vi "Measurement Logic.vi"(8 "error in":errorcluster, 9 "measurement configuration":T2={"Input Terminal Name"="Lorem ipsum dolor sit", "Counter Interface"="", "Active Edge"=10171, "Pulses"=0, "Timeout (s)"=0, "DUT Pin"=""} {"Active Edge" items=["Rising"=10280, "Falling"=10171]}, 10 "measure call context in":refnum<class "Measure Call Context.lvclass">) -> (0 "error out":errorcluster, 1 "Measurements Resuts":T1, 2 "measure call context out":refnum<class "Measure Call Context.lvclass">)   [LabVIEW 2025, in "Count Edges.lvclass"]
doc: "Contains the core logic for executing the measurement."
uses:
  Count Edges.lvclass
  <vilib>/Plug-In SDKs/Measurements/Measure Call Context/Measure Call Context.lvclass
  Measurement Configuration.ctl
  Measurement Results.ctl
  <vilib>/DAQmx/read.llb/DAQmx Read (Counter U32 1Chan 1Samp).vi
  <vilib>/DAQmx/create/channels.llb/DAQmx Create Channel (CI-Count Edges).vi
  <vilib>/DAQmx/miscellaneous.llb/DAQmx Fill In Error Info.vi
  <extravilib>/ChannelInstances/Event Messenger-bool/Instantiate.vi
  <resource>/objmgr/daqmx.rc
  <vilib>/Plug-In SDKs/Clients/Session Management V1/Session Reservation/Session Reservation.lvclass
  session-management/daqmxCounter/Session Management daqmxCounter.lvlib
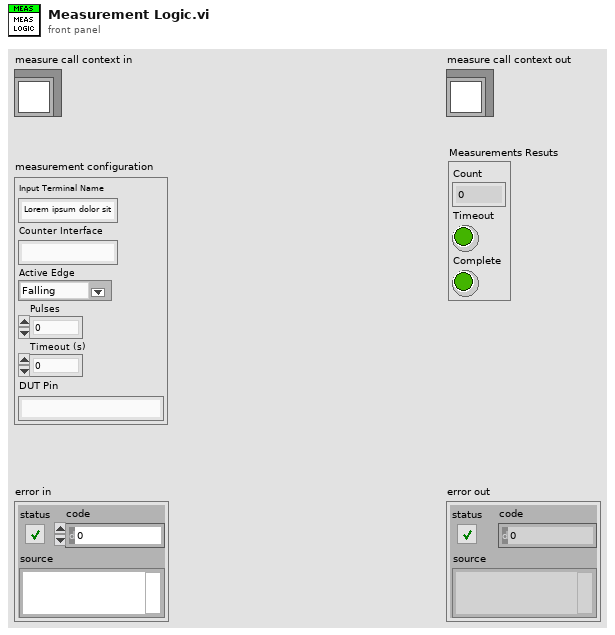
[diagram p1: front panel]
types:
  T1 = typedef "Count Edges.lvclass/Measurement Results.ctl" = cluster{"Count":u32, "Timeout":bool, "Complete":bool}
  T2 = typedef "Count Edges.lvclass/Measurement Configuration.ctl" = cluster{"Input Terminal Name":string, "Counter Interface":string, "Active Edge":i32, "Pulses":u32, "Timeout (s)":u32, "DUT Pin":string}
  T3 = typedef "Session Management daqmxCounter.lvlib/Connection with Session.ctl" = cluster{"connection":T4, "session":string}
  T4 = typedef "NI Session Management V1 Client.lvlib/Session Reservation.lvclass/Connection.ctl" = cluster{"pin or relay name":string, "site":i32, "instrument type id":string, "channel":string}
  T5 = typedef "Event Messenger-bool.lvlib/))Channel.ctl" = refnum<queue>
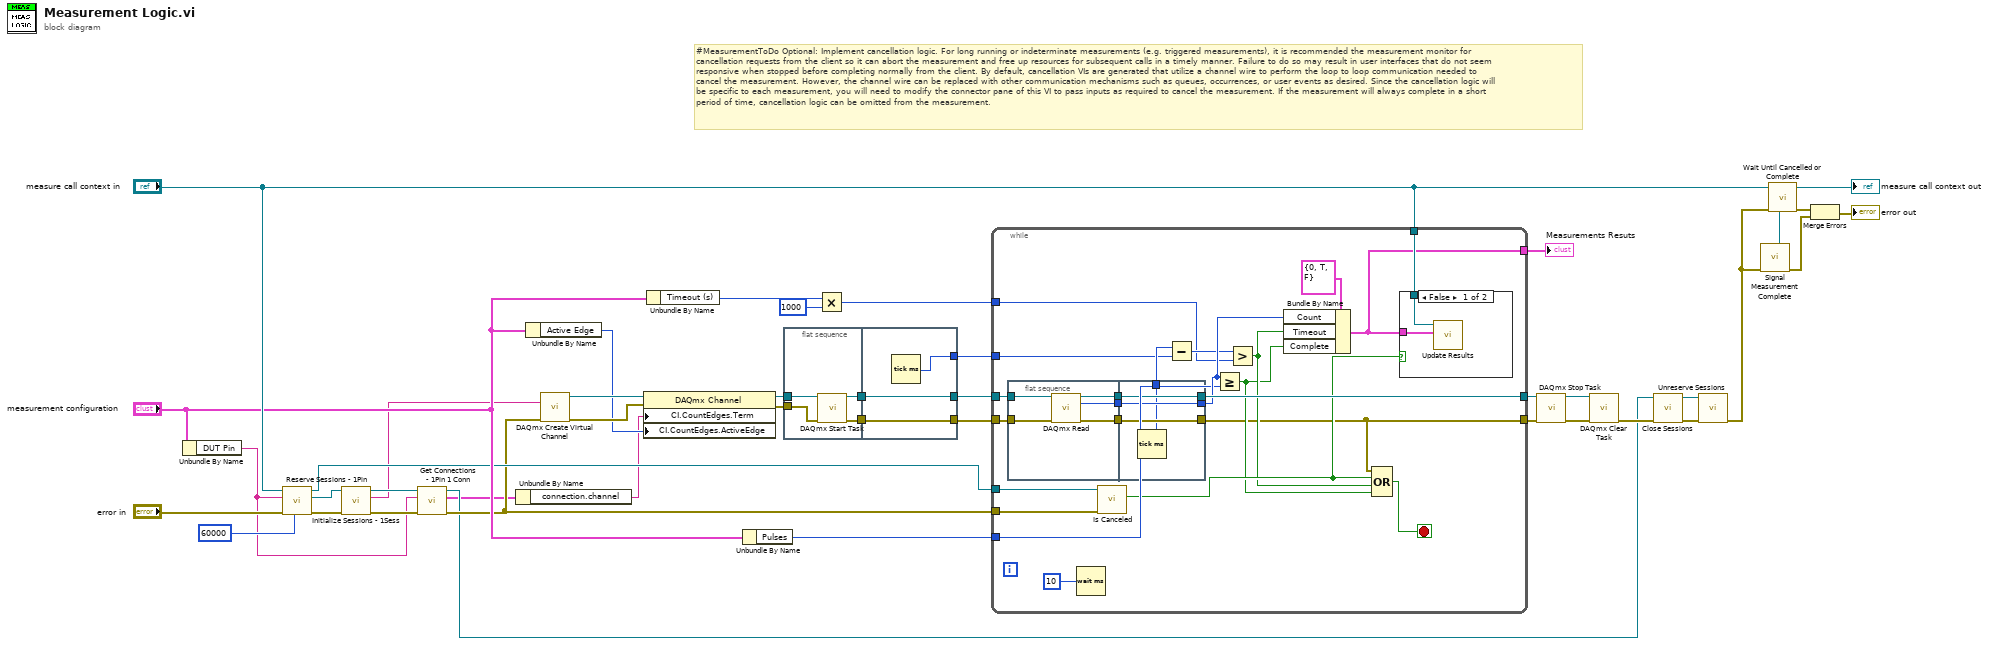
[diagram p0: block diagram]
diagram:
  # "#MeasurementToDo Optional: Implement cancellation logic. For long running or indeterminate measurements (e.g. triggered measurements), it is recommended the measurement monitor for cancellation requests from the client so it can abort the measurement and free up resources for subsequent calls in a timely manner. Failure to do so may result in user interfaces that do not seem responsive when stopped before completing normally from the client. By default, cancellation VIs are generated that utilize a channel wire to perform the loop to loop communication needed to cancel the measurement. However, the channel wire can be replaced with other communication mechanisms such as queues, occurrences, or user events as desired. Since the cancellation logic will be specific to each measurement, you will need to modify the connector pane of this VI to pass inputs as required to cancel the measurement. If the measurement will always complete in a short period of time, cancellation logic can be omitted from the measurement."
  n1 = Unbundle By Name("measurement configuration") -> ("DUT Pin"=w8:string)
  n2 = call <vilib>:"Reserve Sessions - 1Pin.vi"("timeout (ms)"=60000 ("timeout in milliseconds"), "error in"="error in", "pin or relay name"=w8, "measurement context in"="measure call context in") -> ("error out"=w12:errorcluster, "session reservation out"=w13:refnum<class "Session Reservation.lvclass">, "measurement context out"=w11:refnum<class "Measure Call Context.lvclass">)  [unwired: 5 in]
  n3 = call "Initialize Sessions - 1Sess.vi"("error in"=w12, "session reservation in"=w13) -> ("error out"=w9:errorcluster, "session"=w4:string, "session reservation out"=w10:refnum<class "Session Reservation.lvclass">)  [unwired: 6 in, 1 out]
  n4 = call "Get Connections - 1Pin 1 Conn.vi"("error in"=w9, "pin or relay name"=w8, "session reservation in"=w10) -> ("error out"=w7:errorcluster, "connection"=w2:T3, "session reservation out"=w5:refnum<class "Session Reservation.lvclass">)  [unwired: 6 in]
  n5 = Unbundle By Name(w2) -> ("connection.channel"=w1:string)
  n6 = Unbundle By Name("measurement configuration") -> ("Active Edge"=w30:i32)
  n7 = call-poly <vilib>:"DAQmx Create Virtual Channel.vi"("counter"=w4, "error in"=w7) -> ("task out"=w36:refnum<k21>, "error out"=w35:errorcluster)  [unwired: 12 in]
  n8 = property class="DAQmx Channel"(reference=w36, error in=w35, "CI.CountEdges.Term"=w1, "CI.CountEdges.ActiveEdge"=w30) -> (reference out=w21:refnum<k21>, error out=w38:errorcluster)
  n9 = Unbundle By Name("measurement configuration") -> ("Timeout (s)"=w27:u32)
  n10 = Unbundle By Name("measurement configuration") -> ("Pulses"=w29:u32)
  n11 = flat-sequence {
    tunnel: w38 -> [w47]
    tunnel: [w46] -> w25
    tunnel: [w45] -> w24
    tunnel: w21 -> [w44]
    tunnel: [w50] -> w37
    tunnel: w25 -> [w49]
    tunnel: w24 -> [w50]
    tunnel: [w49] -> w23
    tunnel: [w48] -> w22
    frame #0 {
      n12 = call <vilib>:"DAQmx Start Task.vi"("task/channels in"=w44, "error in"=w47) -> ("task out"=w46:refnum<k21>, "error out"=w45:errorcluster)  [unwired: 12 in]
    }
    frame #1 {
      n13 = Tick Count (ms)() -> (millisecond timer value=w48:u32)
    }
  }
  n14 = Multiply(x=w27, y=u32 1000) -> (x*y=w26:u32)
  n15 = while {
    tunnel: w37 -> [w73]
    tunnel: [w51] -> w33
    tunnel: [w72] -> w34
    tunnel: w7 -> [w70]
    tunnel: w11 -> [w69]
    tunnel: w29 -> [w67]
    tunnel: w22 -> [w62]
    tunnel: w26 -> [w60]
    tunnel: w23 -> [w59]
    tunnel: "measure call context in" -> [w57]
    tunnel: [w56] -> w20
    stop <- w52 stop-if-true
    n16 = flat-sequence {
      tunnel: w73 -> [w80]
      tunnel: [w79] -> w66
      tunnel: [w78] -> w65
      tunnel: [w77] -> w64
      tunnel: w59 -> [w76]
      tunnel: [w82] -> w68
      tunnel: [w83] -> w51
      tunnel: [w84] -> w72
      tunnel: w66 -> [w84]
      tunnel: w65 -> [w83]
      tunnel: w64 -> [w82]
      tunnel: [w81] -> w63
      frame #0 {
        n17 = call-poly <vilib>:"DAQmx Read.vi"("task/channels in"=w76, "error in"=w80) -> ("task out"=w79:refnum<k21>, "data"=w77:u32, "error out"=w78:errorcluster)  [unwired: 11 in]
      }
      frame #1 {
        n18 = Tick Count (ms)() -> (millisecond timer value=w81:u32)
      }
    }
    n19 = Wait (ms)(milliseconds to wait=u32 10 ("Loop Time (ms)")) -> ()  [unwired: 1 out]
    n20 = call <vilib>:"Is Canceled.vi"("error in"=w70, "measure call context in"=w69) -> ("is canceled?"=w55:bool)  [unwired: 7 in, 2 out]
    n21 = Subtract(x=w63, y=w62) -> (x-y=w61:u32)
    n22 = Greater Or Equal?(x=w68, y=w67) -> (x >= y?=w53:bool)
    n23 = Greater?(x=w61, y=w60) -> (0:w54:bool)
    n24 = Bundle By Name(cluster=T1 {"Count"=0, "Timeout"=TRUE, "Complete"=FALSE} ("measurement results"), "Count"=w68, "Timeout"=w54, "Complete"=w53) -> (w56:T1)
    n25 = Compound Arithmetic op=OR(w51, w55, w54, w53) -> (w52:bool)
    n26 = case shown="False" w55 {
      tunnel: w56 -> [w75 _]
      tunnel: w57 -> [w74 _]
      frame False {
        n27 = call <vilib>:"Update Results.vi"("measurement results"=w75, "measure call context in"=w74) -> ()  [unwired: 8 in, 2 out]
      }
      frame True {
      }
    }
  }
  "Measurements Resuts" <- w20
  n28 = call <vilib>:"DAQmx Stop Task.vi"("task/channels in"=w34, "error in"=w33) -> ("task out"=w31:refnum<k21>, "error out"=w32:errorcluster)  [unwired: 12 in]
  n29 = call <vilib>:"DAQmx Clear Task.vi"("task in"=w31, "error in"=w32) -> ("error out"=w6:errorcluster)  [unwired: 13 in]
  n30 = call <vilib>:"Close Sessions.vi"("error in"=w6, "session reservation in"=w5) -> ("error out"=w18:errorcluster, "session reservation out"=w17:refnum<class "Session Reservation.lvclass">)  [unwired: 8 in]
  n31 = call <vilib>:"Unreserve Sessions.vi"("error in"=w18, "session reservation in"=w17) -> ("error out"=w3:errorcluster)  [unwired: 9 in]
  n32 = call "Signal Measurement Complete.vi"("error in (no error)"=w3) -> ("error out"=w41:errorcluster, "done channel"=w42:T5)  [unwired: 9 in]
  n33 = call "Wait Until Cancelled or Complete.vi"("done channel"=w42, "error in (no error)"=w3, "measure call context in"="measure call context in") -> ("error out"=w40:errorcluster, "measure call context out"=→"measure call context out":refnum<class "Measure Call Context.lvclass">)  [unwired: 7 in]
  n34 = Merge Errors(w40, w41) -> (→"error out":errorcluster)
